vi "main.vi"() -> ()   [LabVIEW 2023]
uses:
  KYFGLib_lv.lvlib
panel:
  out "IsChameleon":bool=TRUE
  in  "Camera Control":T1(tab)
  in  "GetCameraXML":bool
  out "Camera xml file":string
  out "Camera xml file size":u64
  out "Camera registers read array":u8[](array[numeric]) format="%x"
  in  "Camera register read address":u64 format="%x"
  in  "Camera register read size":u32
  in  "Camera Read Register":bool
  in  "Camera register write address":u64 format="%x"
  in  "Camera Write Register":bool
  in  "Camera register write size":u32
  in  "Camera registers write array":u8[](array[numeric])
  in  "stop":bool
  in  "Playing":bool
  in  "Tab Control":enum32{"Main", "Debug"}(tab)
  in  "Action":bool
  in  "Cameras":u32(ring) items=["0"=131328]
  in  "Frame Grabbers":u32(ring) items=["Chameleon II CXP Camera Simulator", "Komodo CXP Frame Grabber", "KAYA Software Grabber Emulator: CoaXPress (virtual)"]
  out "frame index":i32
  in  "Image Width":u32=1280
  in  "Image Height":u32=720
  out "2D Picture":picture
  out "Connection Mask":string
  out "bufferIndexCurrent":i32
  in  "error in":errorcluster
  out "error out":errorcluster={"status"=FALSE, "code"=12288, "source"=""}
  out "buffHandle":u32
  out "camHandle":u32
  out "buffer size":u64
  out "FG handle":u32=65536
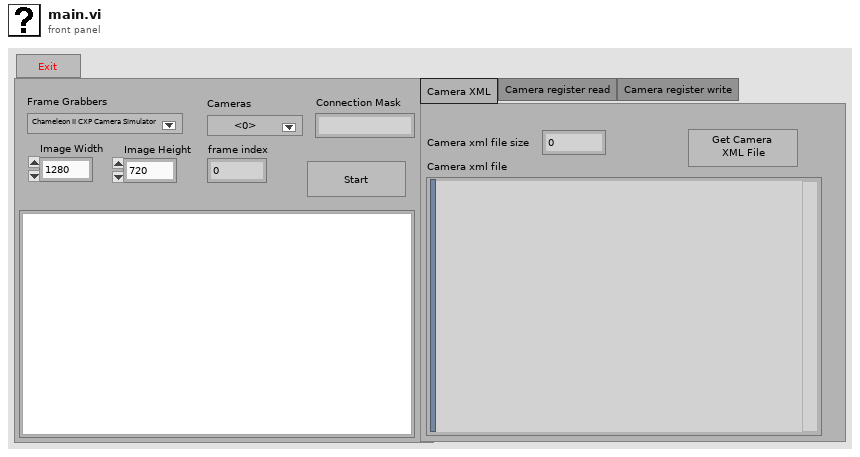
[diagram p1: front panel]
types:
  T1 = enum32{"Camera XML", "Camera register read", "Camera register write"}
  T2 = enum8{"Enabled", "Disabled", "Disabled and Grayed Out"}
  T3 = enum32{"PATTERN_XRAMP", "PATTERN_XRAMP_COLOR", "PATTERN_YRAMP", "PATTERN_YRAMP_COLOR", "PATTERN_XYRAMP", "PATTERN_XYRAMP_COLOR"}
  T4 = typedef "imagedata.ctl" = cluster{"image type":i32, "image depth":i32, "image":u8[], "mask":u8[], "colors":u32[], "Rectangle":cluster{"left":i16, "top":i16, "right":i16, "bottom":i16}}
  T5 = typedef "LVBoundsTypeDef.ctl" = cluster{"Width":u32, "Height":u32}
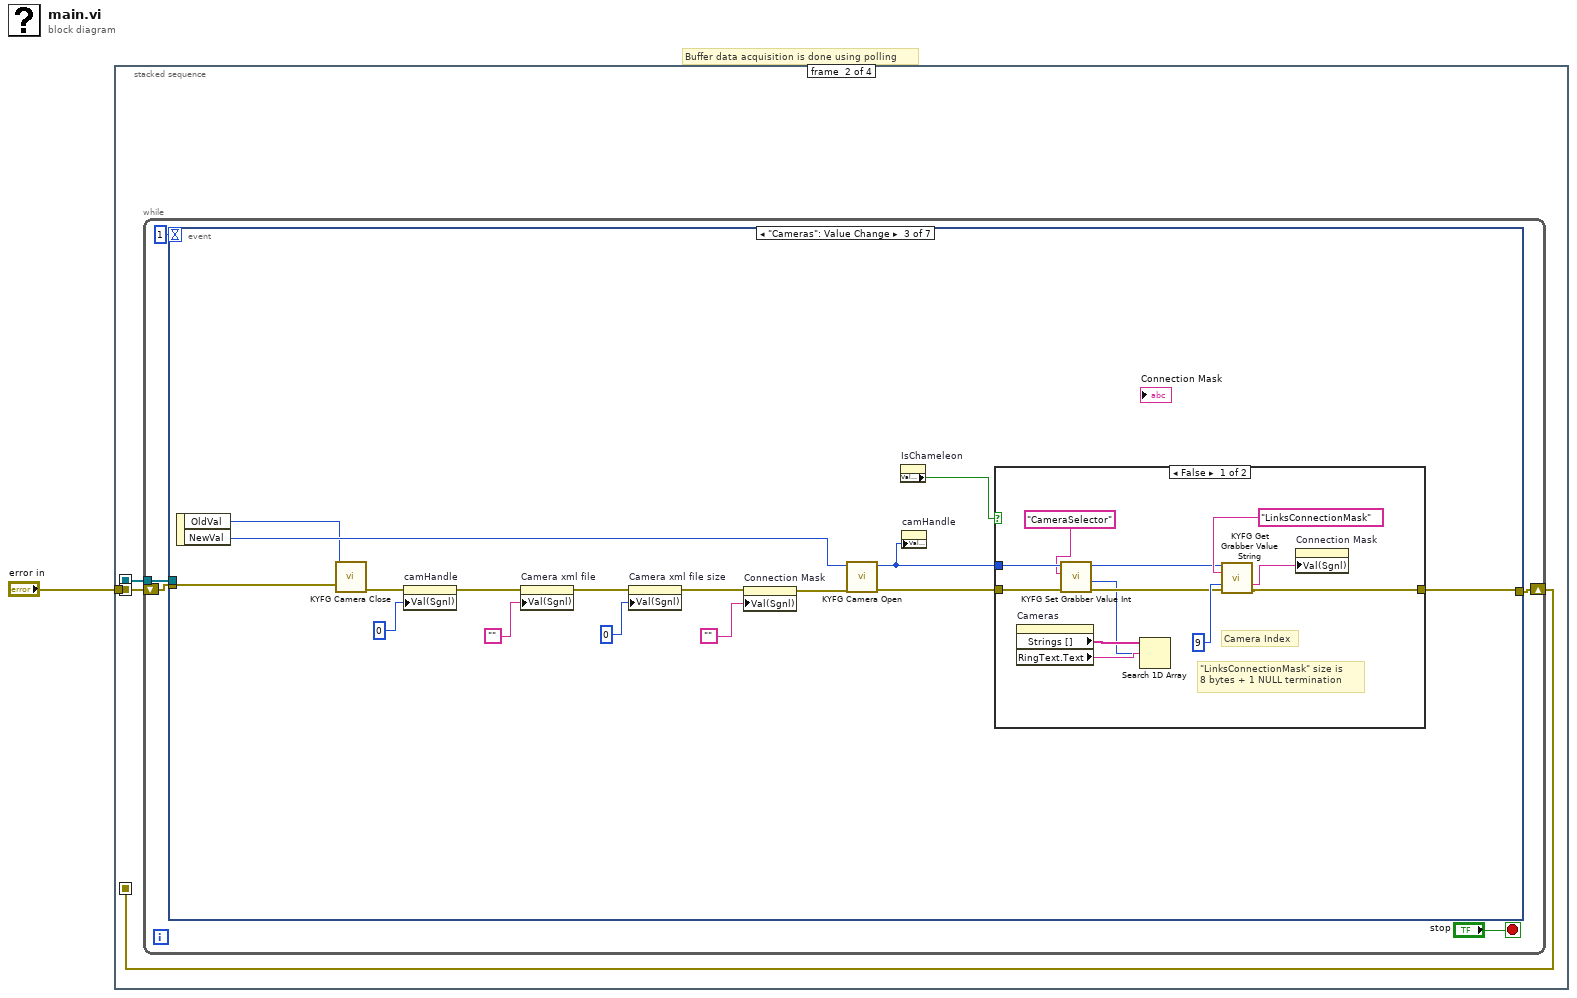
[diagram p0: block diagram]
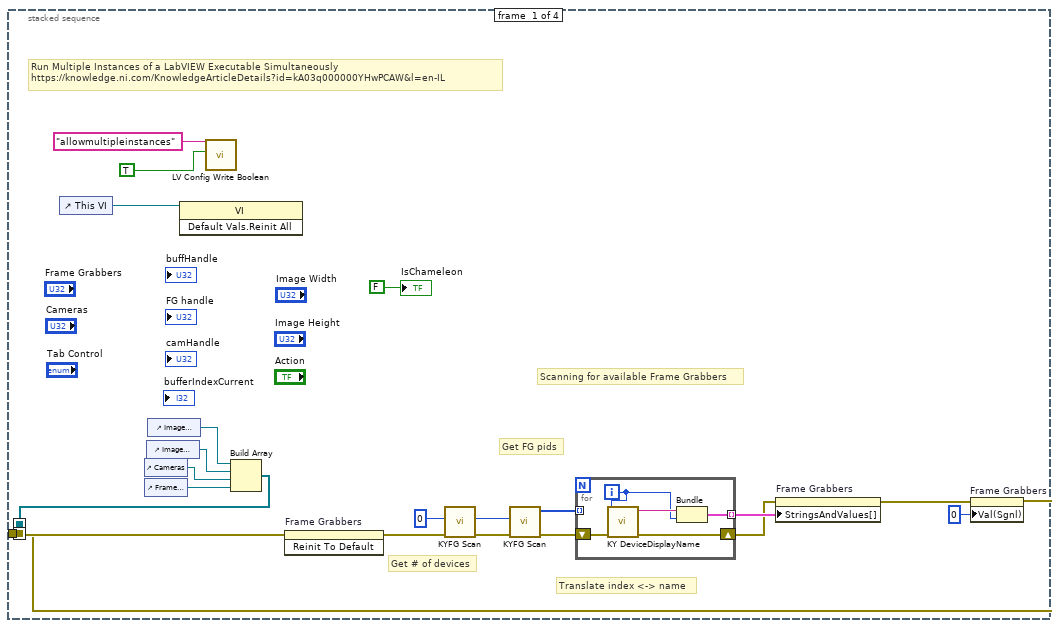
[diagram p2: hidden frame]
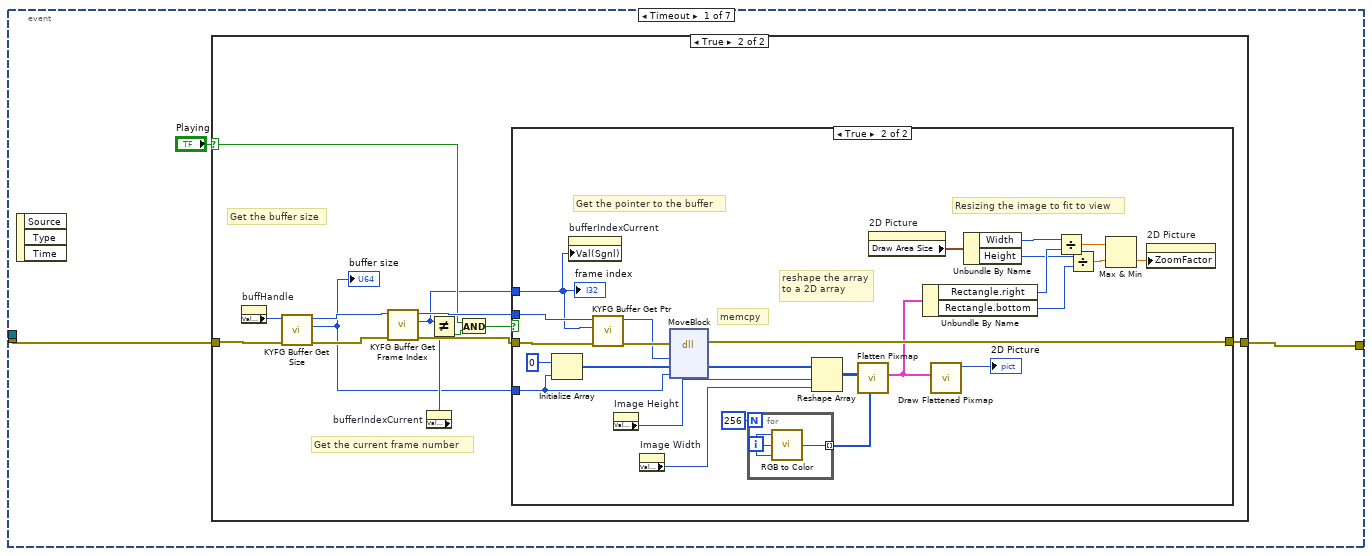
[diagram p3: hidden frame]
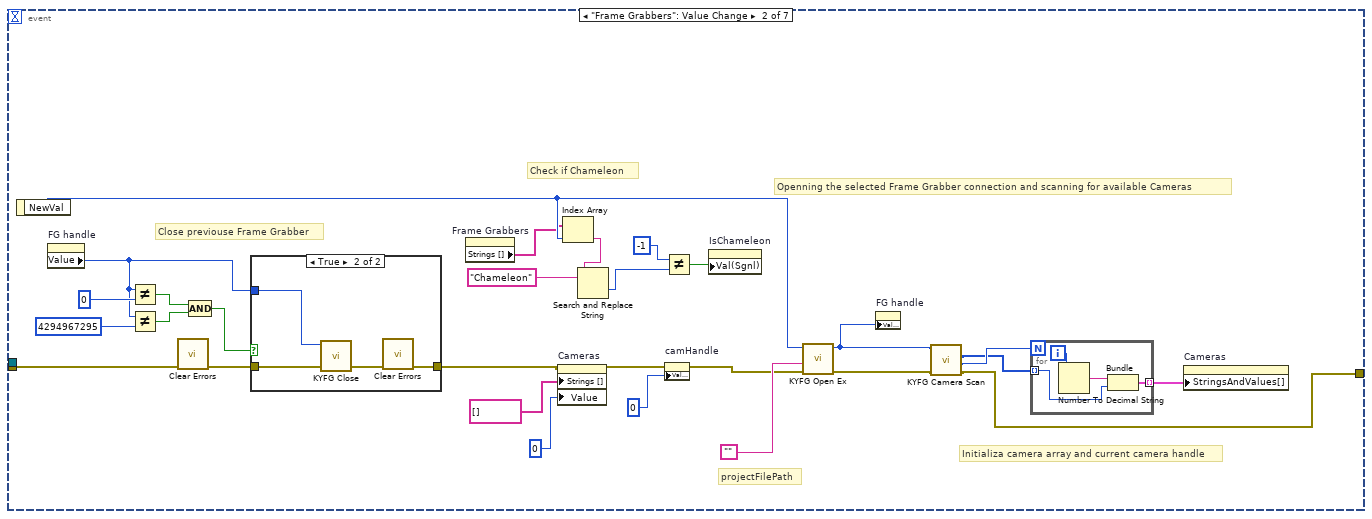
[diagram p6: hidden frame]
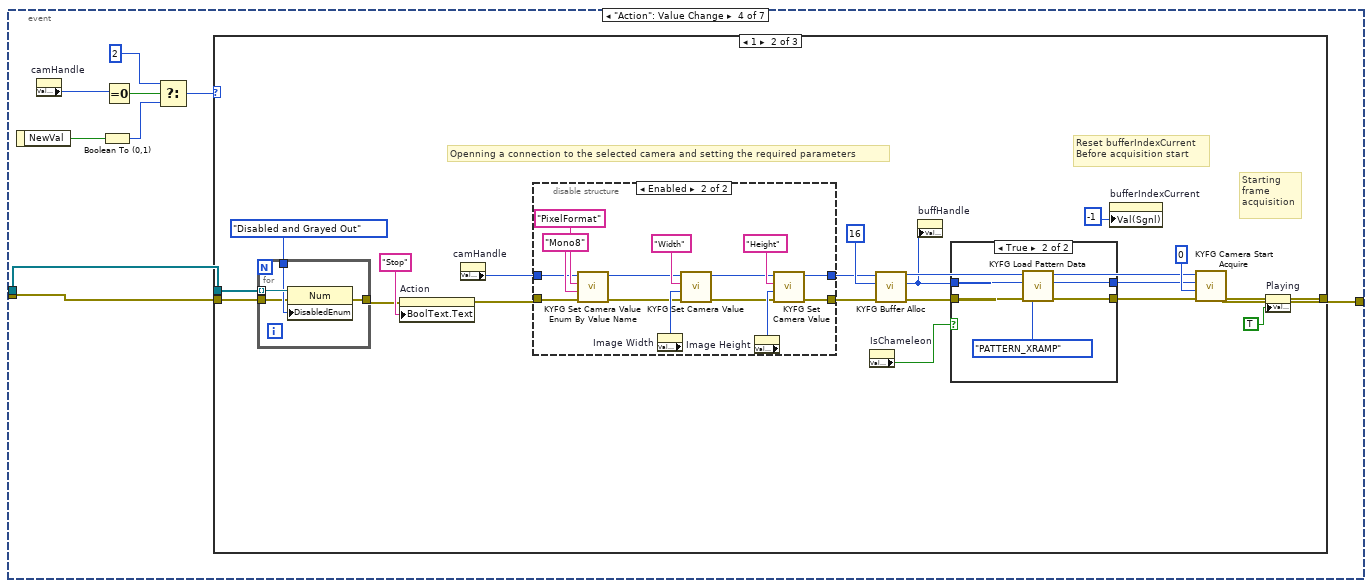
[diagram p9: hidden frame]
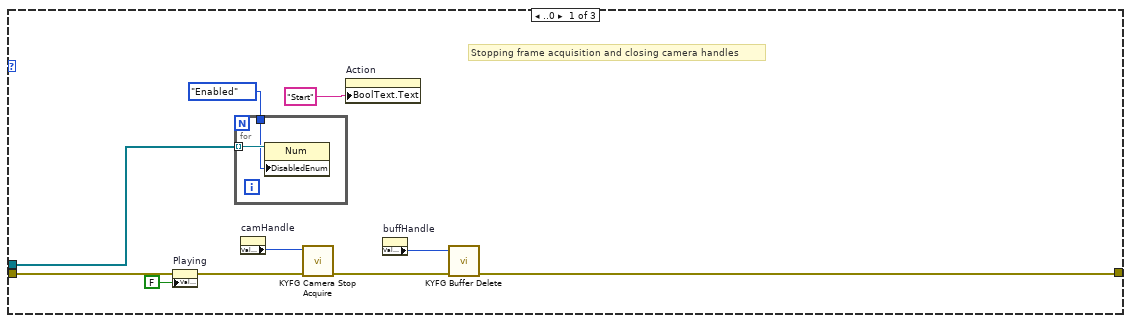
[diagram p10: hidden frame]
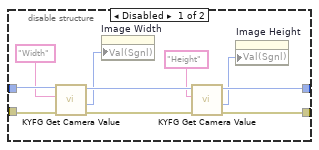
[diagram p12: hidden frame]
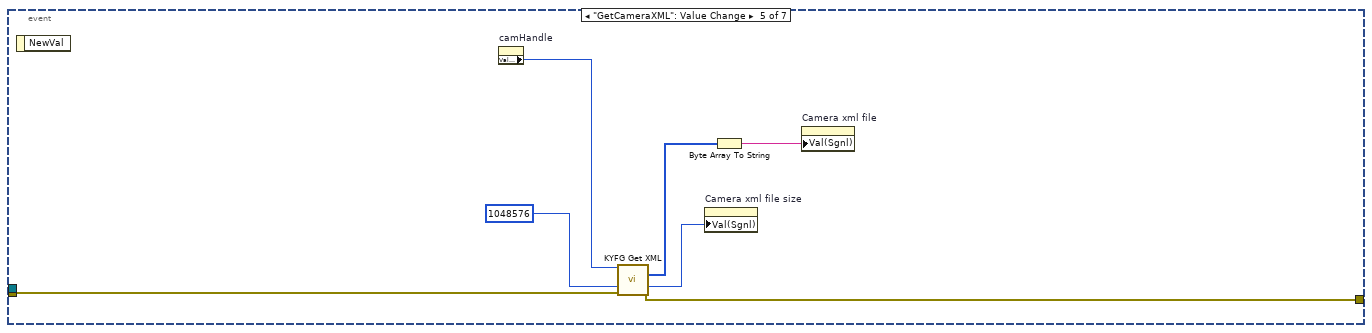
[diagram p14: hidden frame]
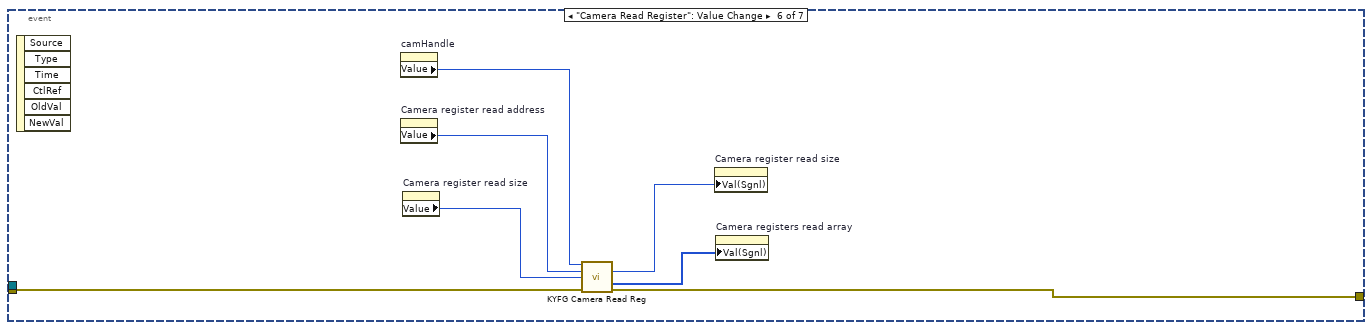
[diagram p15: hidden frame]
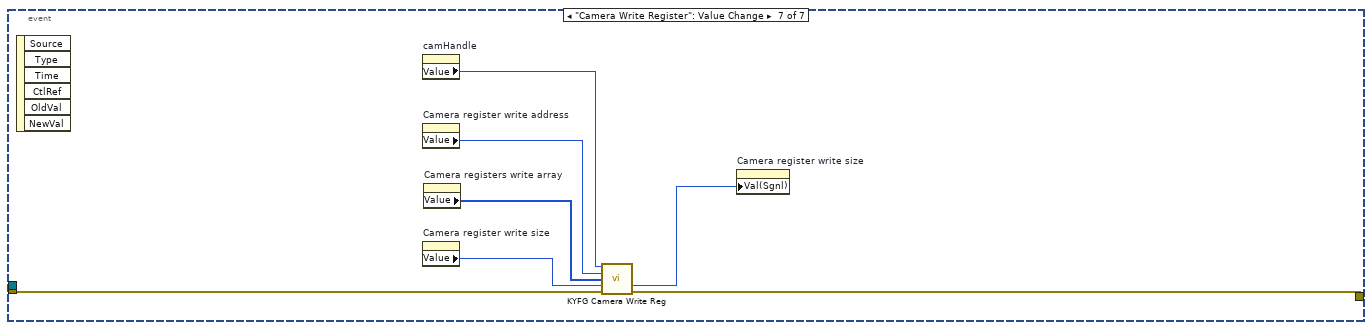
[diagram p16: hidden frame]
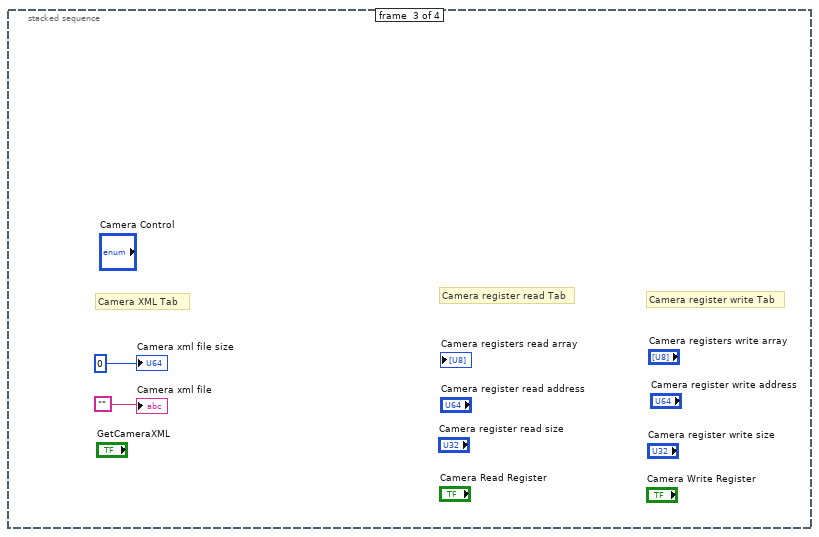
[diagram p17: hidden frame]
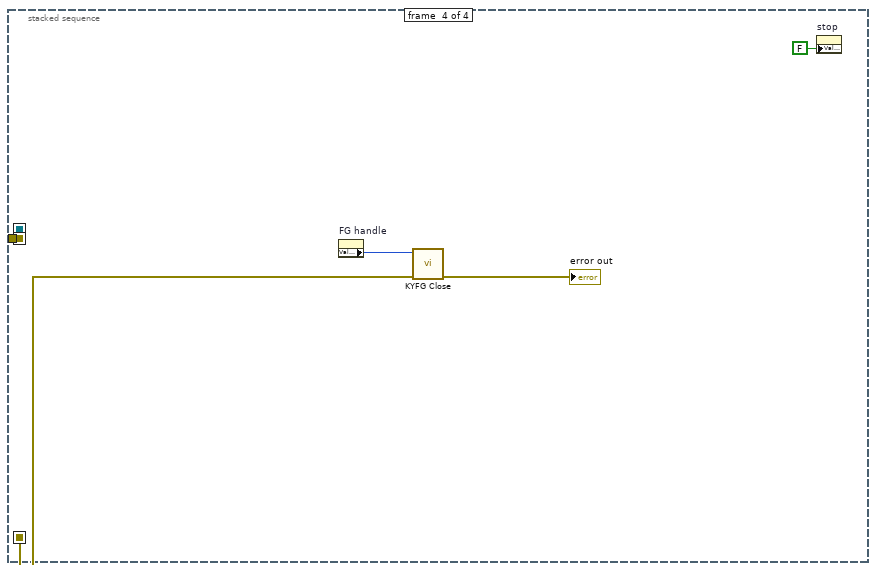
[diagram p18: hidden frame]
diagram:
  # "Buffer data acquisition is done using polling"
  n1 = stacked-sequence {
    seq-local: [w20 _ _ _] -> [_ w30 _ _]
    seq-local: [_ w29 _ _] -> [_ _ _ w250]
    seq-local: [w4 _ _ _] -> [_ w28 _ _]
    tunnel: "error in" -> [w5 _ _ _]
    frame #0 {
      # "Run Multiple Instances of a LabVIEW Executable Simultaneously\nhttps://knowledge.ni.com/KnowledgeArticleDetails?id=kA03q000000YHwPCAW&l=en-IL"
      # "Translate index <-> name"
      # "Scanning for available Frame Grabbers"
      # "Get FG pids"
      # "Get # of devices"
      n2 = control-ref of="This VI"() -> (w8:refnum<vi>)
      n3 = control-ref of="Cameras"() -> (w22:refnum<vi>)
      n4 = control-ref of="Frame Grabbers"() -> (w21:refnum<vi>)
      n5 = control-ref of="Image Height"() -> (w19:refnum<vi>)
      n6 = control-ref of="Image Width"() -> (w18:refnum<vi>)
      n7 = invoke class="VI" method="Default Vals.Reinit All"(reference=w8) -> ()  [unwired: 2 in, 3 out]
      n8 = call <resource>:"LV Config Write Boolean.vi"("value"=TRUE, "key"="allowmultipleinstances") -> ()  [unwired: 5 in, 1 out]
      n9 = Build Array(w18, w19, w22, w21) -> (w20:refnum<vi>[])
      n10 = invoke on="Frame Grabbers" class="Ring (strict)" method="Reinit To Default"(error in=w5) -> (error out=w10:errorcluster)  [unwired: 2 in, 2 out]
      n11 = call "KYFG Scan.vi"("error in (no error)"=w10, "count"=0) -> ("error out"=w15:errorcluster, "infosize"=w16:i32)  [unwired: 7 in, 1 out]
      n12 = call "KYFG Scan.vi"("error in (no error)"=w15, "count"=w16) -> ("error out"=w13:errorcluster, "pids_info"=w14:u32[])  [unwired: 7 in, 1 out]
      n13 = for {
        tunnel: w14 -> [_] mode=indexing
        shift-right: [w26] -> w11
        shift-left: w13 -> [w27]
        tunnel: [w24] -> w12 mode=indexing
        i -> [w23]
        n14 = call "KY DeviceDisplayName.vi"("error in (no error)"=w27, "index"=w23) -> ("error out"=w26:errorcluster, "function return"=w25:string)  [unwired: 8 in]
        n15 = Bundle("function return"=w25, w23) -> (w24:cluster{"function return":string, i32})  [unwired: 1 in]
      }
      n16 = property on="Frame Grabbers" class="Ring (strict)"(error in=w11, "StringsAndValues[]"=w12) -> (error out=w9:errorcluster)  [unwired: 1 in, 1 out]
      n17 = property on="Frame Grabbers" class="Ring (strict)"(error in=w9, "Val(Sgnl)"=0 ("Value (Signaling)")) -> (error out=w4:errorcluster)  [unwired: 1 in, 1 out]
      "IsChameleon" <- FALSE
    }
    frame #1 {
      n18 = while {
        shift-right: [w32] -> w29
        shift-left: w28 -> [w35]
        tunnel: w30 -> [w33]
        stop <- "stop" stop-if-true
        n19 = event shown="[2] \"Cameras\": Value Change" {
          selector: _ -> [_ _ _ _ _ _ _]
          dyn-events: _ -> [_ _ _ _ _ _ _]
          timeout: 1 -> [_ _ _ _ _ _ _]
          tunnel: w35 -> [w37 w97 w133 w155 w226 w238 w245]
          tunnel: [w38 w91 w124 w154 w225 w237 w244] -> w32
          tunnel: w33 -> [_ _ _ w153 _ _ _]
          event Timeout {
            n20 = event-data() -> ()  [unwired: 1 in, 3 out]
            n21 = case shown="True" "Playing" {
              selector: "Playing" -> [_ w45]
              tunnel: w37 -> [w39 w47]
              tunnel: [w39 w46] -> w38
              frame False {
              }
              frame True {
                # "Get the current frame number"
                # "Get the buffer size"
                n22 = property on="buffHandle" class="DigNum (strict)"() -> ("Value"=w48:u32)  [unwired: 2 in, 2 out]
                n23 = call "KYFG Buffer Get Size.vi"("error in (no error)"=w47, "buffHandle"=w48) -> ("error out"=w51:errorcluster, "buffer size"=w41:u64, "buffHandle out"=w52:u32)  [unwired: 7 in]
                "buffer size" <- w41
                n24 = call "KYFG Buffer Get Frame Index.vi"("error in (no error)"=w51, "buffHandle"=w52) -> ("error out"=w49:errorcluster, "frame index"=w43:i32, "buffHandle out"=w50:u32)  [unwired: 7 in]
                n25 = property on="bufferIndexCurrent" class="DigNum (strict)"() -> ("Value"=w44:i32)  [unwired: 2 in, 2 out]
                n26 = Not Equal?(x=w43, y=w44) -> (x != y?=w42:bool)
                n27 = And(x=w45, y=w42) -> (x .and. y?=w40:bool)
                n28 = case shown="True" w40 {
                  tunnel: w50 -> [_ w78]
                  tunnel: w49 -> [w53 w77]
                  tunnel: [w53 w74] -> w46
                  tunnel: w41 -> [_ w54]
                  tunnel: w43 -> [_ w55]
                  frame False {
                  }
                  frame True {
                    # "Resizing the image to fit to view"
                    # "Get the pointer to the buffer"
                    # "reshape the array\nto a 2D array"
                    # "memcpy"
                    n29 = Initialize Array(u8 0 ("I32"), w54) -> (w72:u8[])
                    n30 = property on="bufferIndexCurrent" class="DigNum (strict)"("Val(Sgnl)"=w55) -> ()  [unwired: 2 in, 2 out]
                    n31 = call "KYFG Buffer Get Ptr.vi"("error in (no error)"=w77, "frame"=w55, "buffHandle"=w78) -> ("error out"=w75:errorcluster, "buffer data"=w73:u64)  [unwired: 7 in]
                    n32 = property on="Image Height" class="DigNum (strict)"() -> ("Value"=w69:u32)  [unwired: 2 in, 2 out]
                    n33 = property on="Image Width" class="DigNum (strict)"() -> ("Value"=w68:u32)  [unwired: 2 in, 2 out]
                    n34 = dll-call lib="LabVIEW" fn="MoveBlock"(error in=w75, "src"=w73, "dst"=w72, "size"=w54) -> (error out=w74:errorcluster, "dst"=w71:u8[])  [unwired: 5 in, 1 out]
                    n35 = for {
                      N: 256 -> [_]
                      tunnel: [w79] -> w65 mode=indexing
                      i -> [w80]
                      n36 = call <vilib>:"RGB to Color.vi"("B"=w80, "G"=w80, "R"=w80) -> ("Color"=w79:u32)
                    }
                    n37 = Reshape Array(w71, w69, w68) -> (w66:u8[][])
                    n38 = call <vilib>:"Flatten Pixmap.vi"("colors"=w65, "8-bit pixmap"=w66) -> ("image data"=w63:T4)  [unwired: 9 in]
                    n39 = property on="2D Picture" class="Pict"() -> ("Draw Area Size"=w67:T5)  [unwired: 2 in, 2 out]
                    n40 = Unbundle By Name(w63) -> ("Rectangle.right"=w61:i16, "Rectangle.bottom"=w59:i16)
                    n41 = call <vilib>:"Draw Flattened Pixmap.vi"("image data"=w63) -> ("new picture"=→"2D Picture":picture)  [unwired: 8 in]
                    n42 = Unbundle By Name(w67) -> ("Width"=w62:u32, "Height"=w60:u32)
                    n43 = Divide(x=w62, y=w61) -> (x/y=w58:dbl)
                    n44 = Divide(x=w60, y=w59) -> (x/y=w57:dbl)
                    n45 = Max & Min(x=w58, y=w57) -> (min(x,y)=w56:dbl)  [unwired: 1 out]
                    n46 = property on="2D Picture" class="Pict"("ZoomFactor"=w56) -> ()  [unwired: 2 in, 2 out]
                    "frame index" <- w55
                  }
                }
              }
            }
          }
          event "Frame Grabbers": Value Change {
            # "Check if Chameleon"
            # "Close previouse Frame Grabber"
            # "Initializa camera array and current camera handle"
            # "projectFilePath"
            # "Openning the selected Frame Grabber connection and scanning for available Cameras"
            n47 = event-data() -> ("NewVal"=w86:u32)  [unwired: 1 in]
            n48 = property on="FG handle" class="DigNum (strict)"() -> ("Value"=w100:u32)  [unwired: 2 in, 2 out]
            n49 = Not Equal?(x=w100, y=u32 0) -> (x != y?=w105:bool)
            n50 = Not Equal?(x=w100, y=u32 4294967295) -> (x != y?=w103:bool)
            n51 = call <vilib>:"Clear Errors.vi"("error in (no error)"=w97) -> ("error out"=w98:errorcluster)  [unwired: 5 in, 1 out]
            n52 = Compound Arithmetic op=AND(w105, w103) -> (w104:bool)
            n53 = case shown="True" w104 {
              tunnel: w98 -> [w109 w113]
              tunnel: [w109 w110] -> w95
              tunnel: w100 -> [_ w112]
              frame False {
              }
              frame True {
                n54 = call "KYFG Close.vi"("error in (no error)"=w113, "handle"=w112) -> ("error out"=w111:errorcluster)  [unwired: 8 in, 1 out]
                n55 = call <vilib>:"Clear Errors.vi"("error in (no error)"=w111) -> ("error out"=w110:errorcluster)  [unwired: 5 in, 1 out]
              }
            }
            n56 = property on="Frame Grabbers" class="Ring (strict)"() -> ("Strings []"=w84:string[])  [unwired: 2 in, 2 out]
            n57 = property on="Cameras" class="Ring (strict)"(error in=w95, "Strings []"=string[] [], "Value"=0) -> (error out=w96:errorcluster)  [unwired: 1 in, 1 out]
            n58 = Index Array(array=w84, index=w86) -> (element=w85:string)
            n59 = Search and Replace String(input string=w85, search string="Chameleon") -> (offset past replacement=w83:i32)  [unwired: 6 in, 3 out]
            n60 = Not Equal?(x=-1, y=w83) -> (x != y?=w81:bool)
            n61 = property on="camHandle" class="DigNum (strict)"(error in=w96, "Value"=0) -> (error out=w99:errorcluster)  [unwired: 1 in, 1 out]
            n62 = property on="IsChameleon" class="Bool (strict)"("Val(Sgnl)"=w81) -> ()  [unwired: 2 in, 2 out]
            n63 = call "KYFG Open Ex.vi"("error in (no error)"=w99, "projectFile"="", "index"=w86) -> ("error out"=w92:errorcluster, "handle"=w88:u32)  [unwired: 7 in]
            n64 = property on="FG handle" class="DigNum (strict)"("Value"=w88) -> ()  [unwired: 2 in, 2 out]
            n65 = call "KYFG Camera Scan.vi"("error in (no error)"=w92, "handle"=w88) -> ("error out"=w91:errorcluster, "detectedCameras out"=w90:i32, "camHandleArray"=w89:u32[])  [unwired: 7 in]
            n66 = for {
              N: w90 -> [_]
              tunnel: w89 -> [w116] mode=indexing
              tunnel: [w115] -> w108 mode=indexing
              i -> [w114]
              n67 = Number To Decimal String(number=w114) -> (decimal integer string=w117:string)  [unwired: 1 in]
              n68 = Bundle(w117, w116) -> (w115:cluster{string, u32})  [unwired: 1 in]
            }
            n69 = property on="Cameras" class="Ring (strict)"("StringsAndValues[]"=w108) -> ()  [unwired: 2 in, 2 out]
          }
          event "Cameras": Value Change {
            n70 = event-data() -> ("OldVal"=w131:u32, "NewVal"=w132:u32)  [unwired: 1 in]
            n71 = call "KYFG Camera Close.vi"("error in (no error)"=w133, "camHandle"=w131) -> ("error out"=w127:errorcluster)  [unwired: 9 in]
            n72 = property on="camHandle" class="DigNum (strict)"(error in=w127, "Val(Sgnl)"=u32 0) -> (error out=w126:errorcluster)  [unwired: 1 in, 1 out]
            n73 = property on="Camera xml file" class="Str"(error in=w126, "Val(Sgnl)"="") -> (error out=w130:errorcluster)  [unwired: 1 in, 1 out]
            n74 = property on="Camera xml file size" class="DigNum (strict)"(error in=w130, "Val(Sgnl)"=0) -> (error out=w123:errorcluster)  [unwired: 1 in, 1 out]
            n75 = property on="Connection Mask" class="Str"(error in=w123, "Val(Sgnl)"="") -> (error out=w122:errorcluster)  [unwired: 1 in, 1 out]
            n76 = call "KYFG Camera Open.vi"("error in (no error)"=w122, "camHandle"=w132) -> ("error out"=w119:errorcluster, "camHandle out"=w120:u32)  [unwired: 8 in]
            n77 = property on="IsChameleon" class="Bool (strict)"() -> ("Value"=w118:bool)  [unwired: 2 in, 2 out]
            n78 = property on="camHandle" class="DigNum (strict)"("Value"=w120) -> ()  [unwired: 2 in, 2 out]
            n79 = case shown="False" w118 {
              tunnel: [w145 w146] -> w124
              tunnel: w120 -> [w140 _]
              tunnel: w119 -> [w134 w146]
              frame False {
                # "Camera Index"
                # "\"LinksConnectionMask\" size is \n8 bytes + 1 NULL termination"
                n80 = property on="Cameras" class="Ring (strict)"() -> ("Strings []"=w137:string[], "RingText.Text"=w136:string)  [unwired: 2 in, 2 out]
                n81 = Search 1D Array(1D array=w137, element=w136) -> (index of element=w135:i32)  [unwired: 1 in]
                n82 = call "KYFG Set Grabber Value Int.vi"("error in (no error)"=w134, "value"=w135, "paramName"="CameraSelector", "camHandle"=w140) -> ("error out"=w139:errorcluster, "camHandle out"=w141:u32)  [unwired: 6 in]
                n83 = call "KYFG Get Grabber Value String.vi"("handle"=w141, "paramName"="LinksConnectionMask", "stringSize"=9, "error in (no error)"=w139) -> ("stringValueOut"=w144:string, "error out"=w145:errorcluster)  [unwired: 9 in, 1 out]
                n84 = property on="Connection Mask" class="Str"("Val(Sgnl)"=w144) -> ()  [unwired: 2 in, 2 out]
              }
              frame True {
              }
            }
          }
          event "Action": Value Change {
            n85 = event-data() -> ("NewVal"=w152:bool)  [unwired: 1 in]
            n86 = property on="camHandle" class="DigNum (strict)"() -> ("Value"=w148:u32)  [unwired: 2 in, 2 out]
            n87 = Boolean To (0,1)(Boolean=w152) -> (0, 1=w150:i16)
            n88 = Equal To 0?(x=w148) -> (x = 0?=w149:bool)
            n89 = Select(t=2, s=w149, f=w150) -> (s? t:f=w147:i32)
            n90 = case shown="1" w147 {
              tunnel: w155 -> [w161 w182 w224]
              tunnel: [w157 w178 w224] -> w154
              tunnel: w153 -> [w162 w184 _]
              frame ..0 {
                # "Stopping frame acquisition and closing camera handles"
                n91 = property on="Playing" class="Bool (strict)"(error in=w161, "Value"=FALSE ("Playing")) -> (error out=w160:errorcluster)  [unwired: 1 in, 1 out]
                n92 = for {
                  tunnel: w162 -> [w167] mode=indexing
                  tunnel: T2."Enabled" ("Disabled") -> [w166]
                  n93 = property class="Num"(reference=w167, "DisabledEnum"=w166) -> ()  [unwired: 1 in, 2 out]
                }
                n94 = property on="camHandle" class="DigNum (strict)"() -> ("Value"=w164:u32)  [unwired: 2 in, 2 out]
                n95 = call "KYFG Camera Stop Acquire.vi"("error in (no error)"=w160, "camHandle"=w164) -> ("error out"=w158:errorcluster)  [unwired: 8 in, 1 out]
                n96 = property on="Action" class="Bool (strict)"("BoolText.Text"="Start" ("Label.Text")) -> ()  [unwired: 2 in, 2 out]
                n97 = property on="buffHandle" class="DigNum (strict)"() -> ("Value"=w156:u32)  [unwired: 2 in, 2 out]
                n98 = call "KYFG Buffer Delete.vi"("error in (no error)"=w158, "streamHandle"=w156) -> ("error out"=w157:errorcluster)  [unwired: 9 in]
              }
              frame 1 {
                # "Reset bufferIndexCurrent\nBefore acquisition start"
                # "Starting\nframe \nacquisition"
                # "Openning a connection to the selected camera and setting the required parameters"
                n99 = for {
                  tunnel: w184 -> [w223] mode=indexing
                  tunnel: T2."Disabled and Grayed Out" ("Disabled") -> [w222]
                  tunnel: w182 -> [w221]
                  tunnel: [w220] -> w181
                  n100 = property class="Num"(reference=w223, error in=w221, "DisabledEnum"=w222) -> (error out=w220:errorcluster)  [unwired: 1 out]
                }
                n101 = property on="Action" class="Bool (strict)"(error in=w181, "BoolText.Text"="Stop" ("Label.Text")) -> (error out=w175:errorcluster)  [unwired: 1 in, 1 out]
                n102 = property on="camHandle" class="DigNum (strict)"() -> ("Value"=w174:u32)  [unwired: 2 in, 2 out]
                n103 = disable-structure shown="Enabled" {
                  disable-tunnel: [w204 w209] -> w177
                  disable-tunnel: [w200 w208] -> w176
                  disable-tunnel: w175 -> [w202 w207]
                  disable-tunnel: w174 -> [w203 w206]
                  frame Disabled {
                    n104 = call "KYFG Get Camera Value.vi"("error in (no error)"=w202, "paramName"="Width", "camHandle"=w203) -> ("error out"=w201:errorcluster, "paramValue"=w197:i64, "camHandle out"=w205:u32)  [unwired: 6 in]
                    n105 = property on="Image Width" class="DigNum (strict)"("Val(Sgnl)"=w197) -> ()  [unwired: 2 in, 2 out]
                    n106 = call "KYFG Get Camera Value.vi"("error in (no error)"=w201, "paramName"="Height", "camHandle"=w205) -> ("error out"=w200:errorcluster, "paramValue"=w196:i64, "camHandle out"=w204:u32)  [unwired: 6 in]
                    n107 = property on="Image Height" class="DigNum (strict)"("Val(Sgnl)"=w196) -> ()  [unwired: 2 in, 2 out]
                  }
                  frame Enabled {
                    n108 = call "KYFG Set Camera Value Enum By Value Name.vi"("error in (no error)"=w207, "paramValueName"="Mono8", "paramName"="PixelFormat", "camHandle"=w206) -> ("error out"=w212:errorcluster, "camHandle out"=w213:u32)  [unwired: 6 in]
                    n109 = property on="Image Width" class="DigNum (strict)"() -> ("Value"=w219:u32)  [unwired: 2 in, 2 out]
                    n110 = call "KYFG Set Camera Value.vi"("error in (no error)"=w212, "paramValue"=w219, "paramName"="Width", "camHandle"=w213) -> ("error out"=w215:errorcluster, "camHandle out"=w214:u32)  [unwired: 6 in]
                    n111 = property on="Image Height" class="DigNum (strict)"() -> ("Value"=w218:u32)  [unwired: 2 in, 2 out]
                    n112 = call "KYFG Set Camera Value.vi"("error in (no error)"=w215, "paramValue"=w218, "paramName"="Height", "camHandle"=w214) -> ("error out"=w208:errorcluster, "camHandle out"=w209:u32)  [unwired: 6 in]
                  }
                }
                n113 = property on="IsChameleon" class="Bool (strict)"() -> ("Value"=w168:bool)  [unwired: 2 in, 2 out]
                n114 = call "KYFG Buffer Alloc.vi"("error in (no error)"=w176, "frames"=u32 16, "camHandle"=w177) -> ("error out"=w172:errorcluster, "buffHandle"=w170:u32, "camHandle out"=w186:u32)  [unwired: 6 in]
                n115 = property on="buffHandle" class="DigNum (strict)"("Value"=w170) -> ()  [unwired: 2 in, 2 out]
                n116 = case shown="True" w168 {
                  tunnel: w172 -> [w190 w195]
                  tunnel: [w190 w194] -> w171
                  tunnel: w170 -> [w189 w193]
                  tunnel: [w189 w192] -> w169
                  frame False {
                  }
                  frame True {
                    n117 = call "KYFG Load Pattern Data.vi"("error in (no error)"=w195, "patternType"=T3."PATTERN_XRAMP", "streamHandle"=w193) -> ("error out"=w194:errorcluster, "streamHandle out"=w192:u32)  [unwired: 7 in]
                  }
                }
                n118 = property on="bufferIndexCurrent" class="DigNum (strict)"("Val(Sgnl)"=-1) -> ()  [unwired: 2 in, 2 out]
                n119 = call "KYFG Camera Start Acquire.vi"("error in (no error)"=w171, "frames"=u32 0, "buffHandle"=w169, "camHandle"=w186) -> ("error out"=w179:errorcluster)  [unwired: 5 in, 2 out]
                n120 = property on="Playing" class="Bool (strict)"(error in=w179, "Value"=TRUE ("Playing")) -> (error out=w178:errorcluster)  [unwired: 1 in, 1 out]
              }
              frame 2.. {
              }
            }
          }
          event "GetCameraXML": Value Change {
            n121 = event-data() -> ()  [unwired: 1 in, 1 out]
            n122 = property on="camHandle" class="DigNum (strict)"() -> ("Value"=w229:u32)  [unwired: 2 in, 2 out]
            n123 = call "KYFG Get XML.vi"("camHandle"=w229, "bufferSize"=1048576, "error in (no error)"=w226) -> ("buffer"=w228:u8[], "bufferSize out"=w230:u64, "error out"=w225:errorcluster)  [unwired: 8 in, 2 out]
            n124 = property on="Camera xml file size" class="DigNum (strict)"("Val(Sgnl)"=w230) -> ()  [unwired: 2 in, 2 out]
            n125 = Byte Array To String(unsigned byte array=w228) -> (string=w227:string)
            n126 = property on="Camera xml file" class="Str"("Val(Sgnl)"=w227) -> ()  [unwired: 2 in, 2 out]
          }
          event "Camera Read Register": Value Change {
            n127 = event-data() -> ()  [unwired: 1 in, 6 out]
            n128 = property on="camHandle" class="DigNum (strict)"() -> ("Value"=w236:u32)  [unwired: 2 in, 2 out]
            n129 = property on="Camera register read address" class="DigNum (strict)"() -> ("Value"=w234:u64)  [unwired: 2 in, 2 out]
            n130 = property on="Camera register read size" class="DigNum (strict)"() -> ("Value"=w233:u32)  [unwired: 2 in, 2 out]
            n131 = call "KYFG Camera Read Reg.vi"("camHandle"=w236, "address"=w234, "size"=w233, "error in (no error)"=w238) -> ("size out"=w235:u32, "data out"=w232:u8[], "error out"=w237:errorcluster)  [unwired: 8 in, 1 out]
            n132 = property on="Camera register read size" class="DigNum (strict)"("Val(Sgnl)"=w235) -> ()  [unwired: 2 in, 2 out]
            n133 = property on="Camera registers read array" class="Arr (strict)"("Val(Sgnl)"=w232) -> ()  [unwired: 2 in, 2 out]
          }
          event "Camera Write Register": Value Change {
            n134 = event-data() -> ()  [unwired: 1 in, 6 out]
            n135 = property on="camHandle" class="DigNum (strict)"() -> ("Value"=w243:u32)  [unwired: 2 in, 2 out]
            n136 = property on="Camera register write address" class="DigNum (strict)"() -> ("Value"=w240:u64)  [unwired: 2 in, 2 out]
            n137 = property on="Camera register write size" class="DigNum (strict)"() -> ("Value"=w242:u32)  [unwired: 2 in, 2 out]
            n138 = property on="Camera registers write array" class="Arr (strict)"() -> ("Value"=w241:u8[])  [unwired: 2 in, 2 out]
            n139 = call "KYFG Camera Write Reg.vi"("camHandle"=w243, "address"=w240, "data"=w241, "size"=w242, "error in (no error)"=w245) -> ("size out"=w239:u32, "error out"=w244:errorcluster)  [unwired: 8 in, 1 out]
            n140 = property on="Camera register write size" class="DigNum (strict)"("Val(Sgnl)"=w239) -> ()  [unwired: 2 in, 2 out]
          }
        }
      }
    }
    frame #2 {
      # "Camera register write Tab"
      # "Camera XML Tab"
      # "Camera register read Tab"
      "Camera xml file size" <- u64 0 ("Camera xml file size")
      "Camera xml file" <- ""
    }
    frame #3 {
      n141 = property on="FG handle" class="DigNum (strict)"() -> ("Value"=w248:u32)  [unwired: 2 in, 2 out]
      n142 = call "KYFG Close.vi"("error in (no error)"=w250, "handle"=w248) -> ("error out"=→"error out":errorcluster)  [unwired: 8 in, 1 out]
      n143 = property on="stop" class="Bool (strict)"("Value"=FALSE ("stop")) -> ()  [unwired: 2 in, 2 out]
    }
  }
